vi "Prepare Control.vi"(7 "VolatusAPI":refnum<class "VolatusAPI.lvclass">, 8 "error in (no error)":errorcluster, 11 "ValveControl in":refnum<class "DiscreteRangeControl.lvclass">) -> (0 "error out":errorcluster, 3 "ValveControl out":refnum<class "DiscreteRangeControl.lvclass">)   [LabVIEW 2020, in "VolatusControl.lvlib" / "DiscreteRangeControl.lvclass"]
uses:
  DiscreteRangeControl.lvclass
  Volatus/VolatusAPI/VolatusAPI.lvclass
  DiscreteRangeControl.lvclass/DiscreteRangeControl.ctl
  PV Calc/PV Calc.lvclass
  lv-cdm/CDM-Config/Config Element/Config Element.lvclass
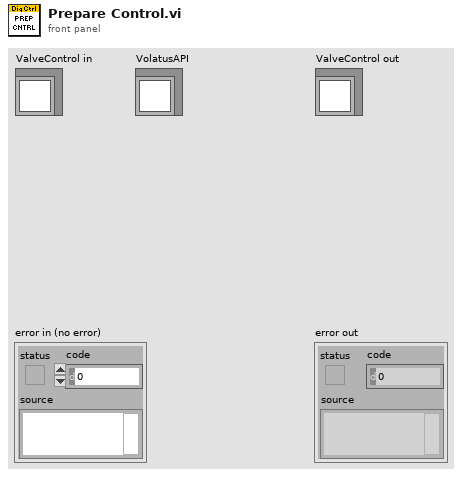
[diagram p1: front panel]
types:
  T1 = typedef "VolatusControl.lvlib/Control Action.ctl" = cluster{"Channel":string, "MsgQ":refnum<class "MessageQ.lvclass">, "Value":bool}
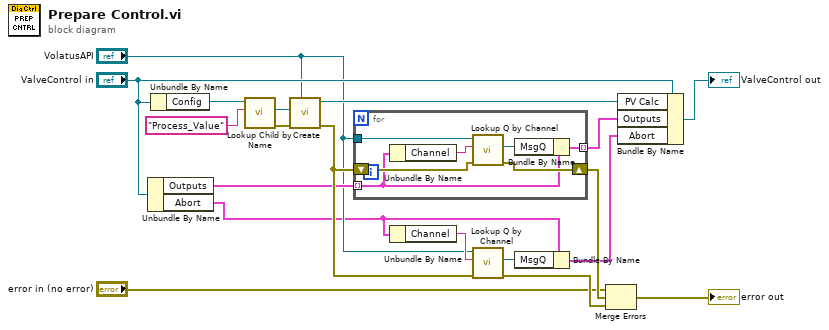
[diagram p0: block diagram]
diagram:
  n1 = Unbundle By Name("ValveControl in") -> ("Outputs"=w11:T1[], "Abort"=w6:T1)
  n2 = Unbundle By Name("ValveControl in") -> ("Config"=w18:refnum<class "Config Element.lvclass">)
  n3 = call "Lookup Child by Name.vi"("Name"="Process_Value", "Config Element in"=w18) -> ("error out"=w13:errorcluster, "Child"=w15:refnum<class "Config Element.lvclass">)  [unwired: 6 in, 2 out]
  n4 = call "Create.vi"("VolatusAPI"="VolatusAPI", "error in (no error)"=w13, "Config Element"=w15) -> ("error out"=w19:errorcluster, "PV Calc out"=w16:refnum<class "PV Calc.lvclass">)  [unwired: 7 in]
  n5 = for {
    tunnel: "VolatusAPI" -> [w24]
    tunnel: w11 -> [w22] mode=indexing
    tunnel: [w20] -> w10 mode=indexing
    shift-right: [w25] -> w5
    shift-left: w19 -> [w26]
    n6 = Unbundle By Name(w22) -> ("Channel"=w23:string)
    n7 = call "Lookup Q by Channel.vi"("error in (no error)"=w26, "Channel Name"=w23, "VolatusAPI in"=w24) -> ("error out"=w25:errorcluster, "MessageQ"=w21:refnum<class "MessageQ.lvclass">)  [unwired: 6 in, 1 out]
    n8 = Bundle By Name(cluster=w22, "MsgQ"=w21) -> (w20:T1)
  }
  n9 = Unbundle By Name(w6) -> ("Channel"=w9:string)
  n10 = call "Lookup Q by Channel.vi"("error in (no error)"=w19, "Channel Name"=w9, "VolatusAPI in"="VolatusAPI") -> ("error out"=w4:errorcluster, "MessageQ"=w8:refnum<class "MessageQ.lvclass">)  [unwired: 6 in, 1 out]
  n11 = Bundle By Name(cluster=w6, "MsgQ"=w8) -> (w3:T1)
  n12 = Merge Errors("error in (no error)", w5, w4) -> (→"error out":errorcluster)
  n13 = Bundle By Name(cluster="ValveControl in", "PV Calc"=w16, "Outputs"=w10, "Abort"=w3) -> (→"ValveControl out":refnum<class "DiscreteRangeControl.lvclass">)
